vi "Playground_Variant Attributes to Cluster.vi"() -> ()   [LabVIEW 2019]
uses:
  Classes/Settings/ObjectSettings/ObjectSettings.lvclass
  subVIs/typedefs/Schedule Types/Schedule--Ramp.ctl
  <vilib>/JDP Science/JSONtext/JSONtext.lvlib
  60cf58b4-a140-46e7-9bca-05715a14d1c5.vi
  26d5b9b7-31bc-4fce-ba1d-d7f4b91fb41a.vi
  subVIs/typedefs/Schedule Types/Schedule--Constant.ctl
  6ec7998a-a771-46c5-871c-0acc70d3b499.vi
  8034bc6a-2b88-43b4-ab5e-da1cf6f0a6e7.vi
panel:
  out "<JSON> 4":string
  out "Data out":T1={"Value"=10.0}
  in  "error in (no error)":errorcluster
  in  "LUT In":variant
  out "<JSON> 2":string caption="<JSON>First JSON Value"
  out "Rest of Input String":string
  out "<JSON> 3":string caption="<JSON>"
  out "names":string[](array[string])
  out "data":string[](array[string])
  out "<JSON>":string
  out "Array":variant[](array[variant])
  out "x/y":dbl
  # "Read"
  # "JDP: 4.65363E-5"
  # "JKI: 0.0002399"
  # "Write"
  # "JDP: 3.40146E-5\nJKI: 8.64174E-5"
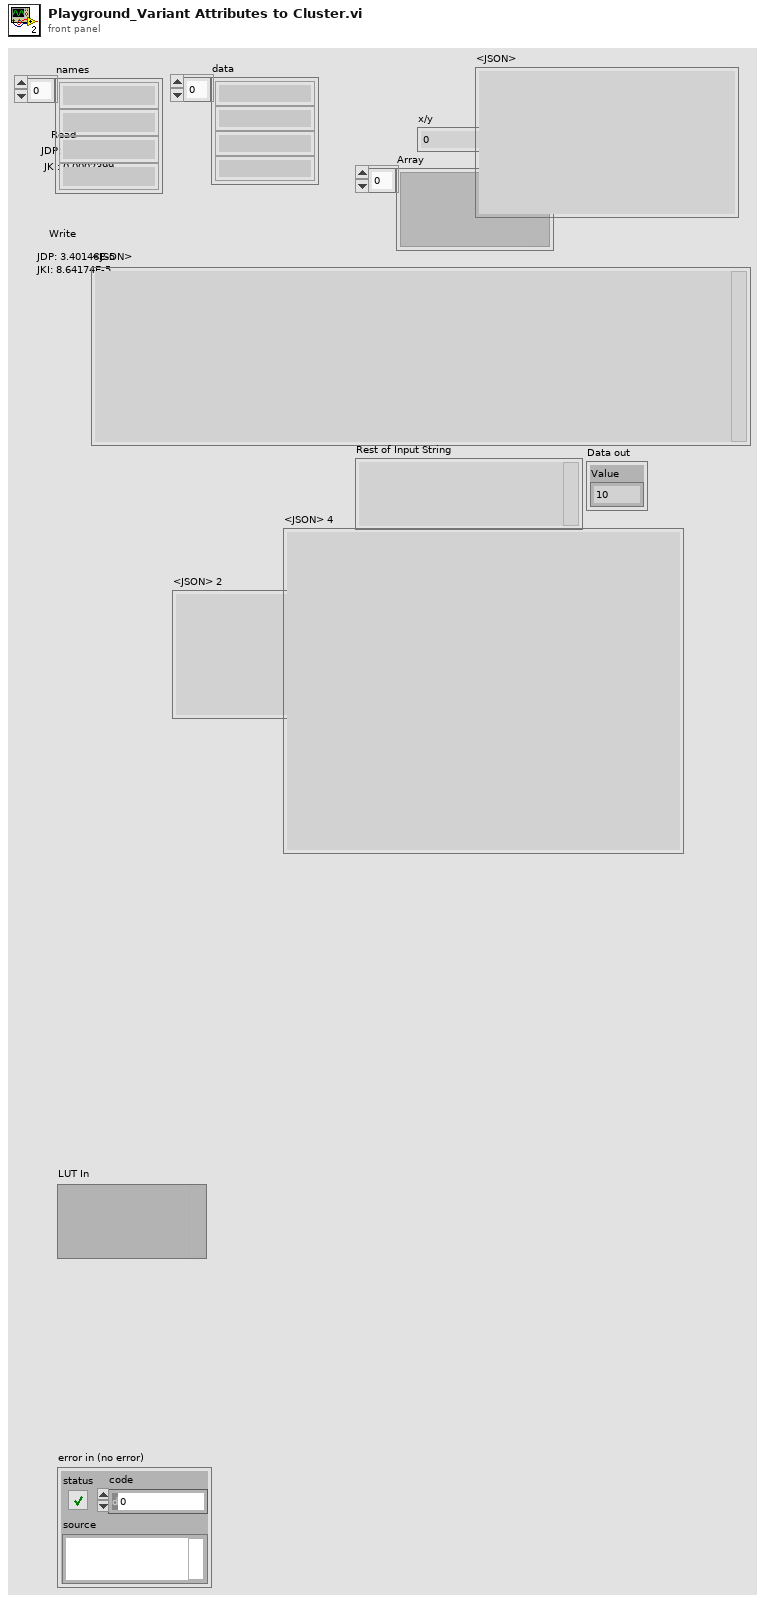
[diagram p1: front panel]
types:
  T1 = typedef "Schedule--Constant.ctl" = cluster{"Value":dbl}
  T2 = typedef "Schedule--Ramp.ctl" = cluster{"Start":dbl, "End":dbl}
  T3 = cluster{"Attribute 1":bool, "Attribute 2":string, "Attribute 3":string}
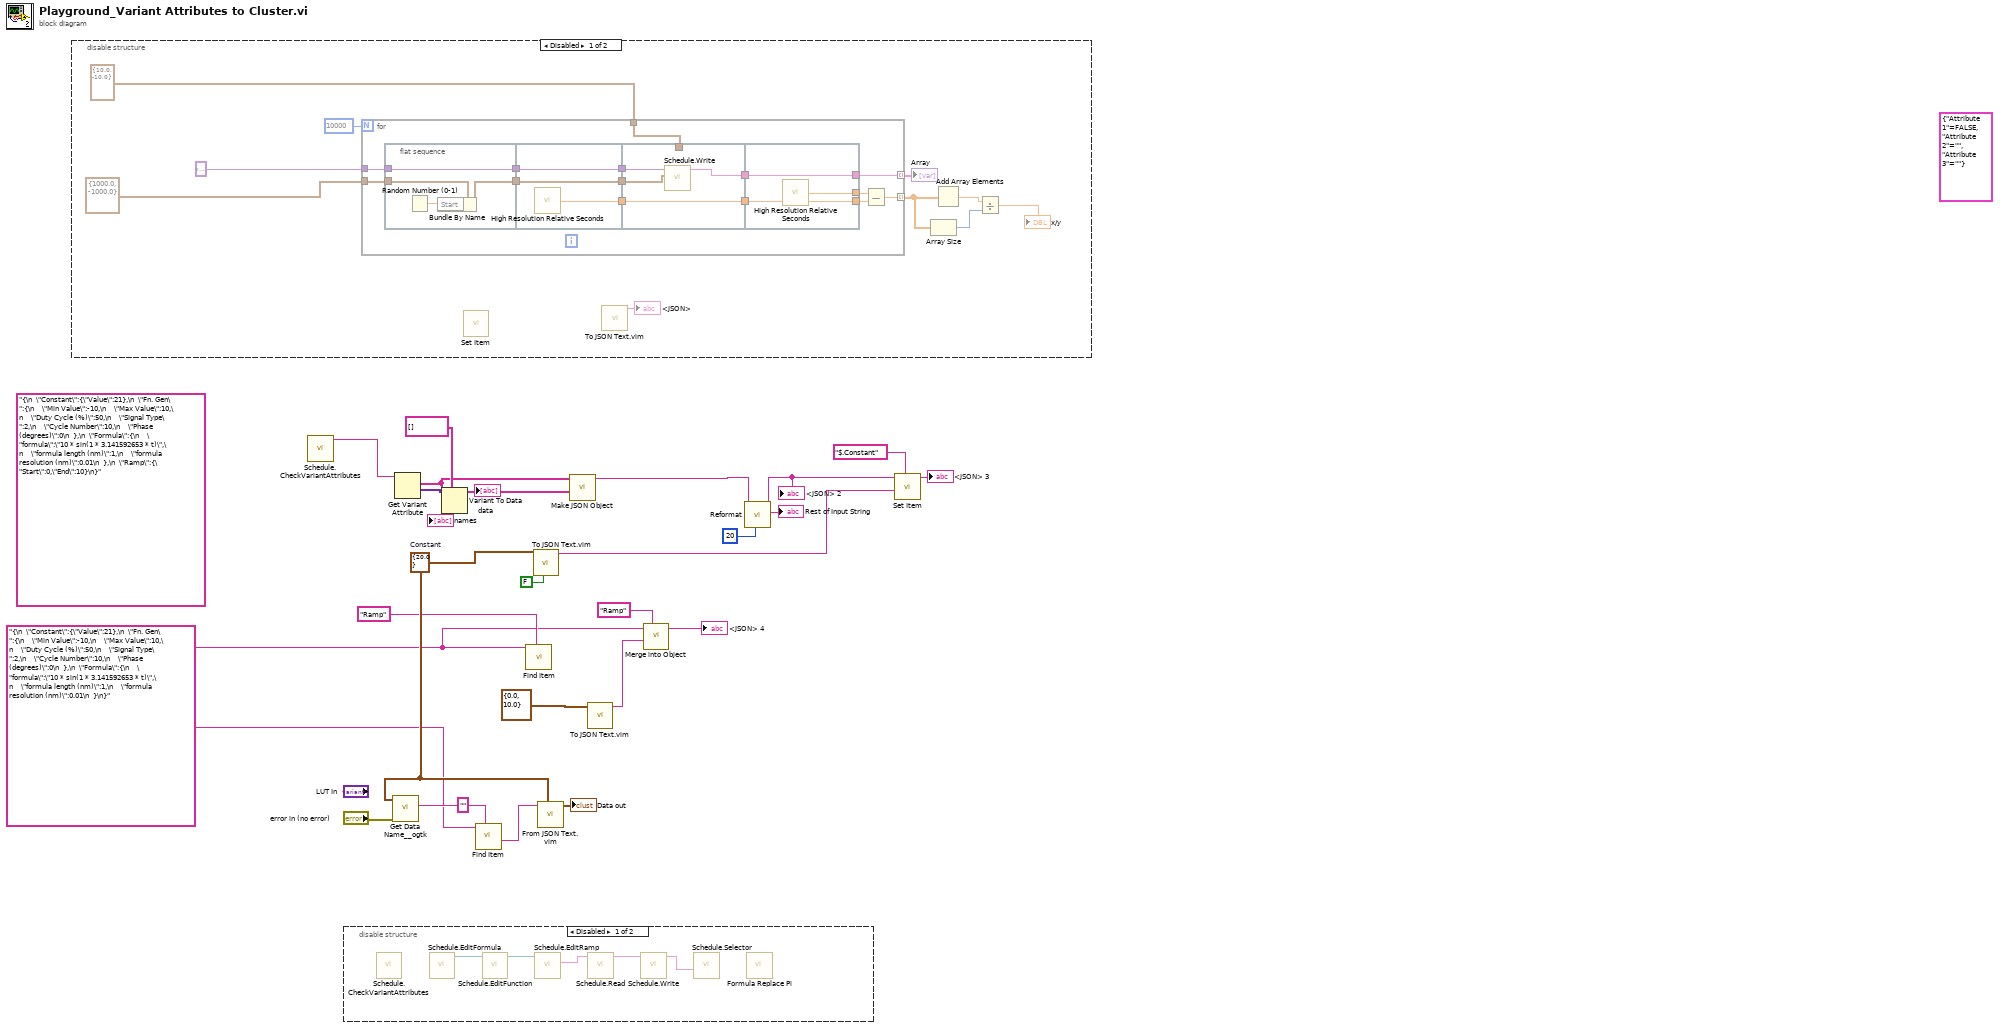
[diagram p0: block diagram]
diagram:
  (unwired) "{\n  \"Constant\":{\"Value\":21},\n  \"Fn. Gen\":{\n    \"Min Value\":-10,\n    \"Max Value\":10,\n    \"Duty Cycle (%)\":50,\n    \"Signal Type\":2,\n    \"Cycle Number\":10,\n    \"Phase (degrees)\":0\n  },\n  \"Formula\":{\n    \"formula\":\"10 * sin(1 * 3.141592653 * t)\",\n    \"formula length (nm)\":1,\n    \"formula resolution (nm)\":0.01\n  },\n  \"Ramp\":{\"Start\":0,\"End\":10}\n}" ("<JSON> 2")
  w4 = "{\n  \"Constant\":{\"Value\":21},\n  \"Fn. Gen\":{\n    \"Min Value\":-10,\n    \"Max Value\":10,\n    \"Duty Cycle (%)\":50,\n    \"Signal Type\":2,\n    \"Cycle Number\":10,\n    \"Phase (degrees)\":0\n  },\n  \"Formula\":{\n    \"formula\":\"10 * sin(1 * 3.141592653 * t)\",\n    \"formula length (nm)\":1,\n    \"formula resolution (nm)\":0.01\n  }\n}" ("<JSON> 2")
  (unwired) ""
  w10 = T1 {"Value"=20.0}  # Constant
  (unwired) T3 {"Attribute 1"=FALSE, "Attribute 2"="", "Attribute 3"=""}
  n1 = disable-structure shown="Disabled" {
    frame Disabled {
      n2 = for {
        N: 10000 -> [_]
        tunnel: T2 {"Start"=10.0, "End"=-10.0} ("Ramp") -> [w47]
        tunnel: variant ("LUT In") -> [w49]
        tunnel: [w48] -> w27 mode=indexing
        tunnel: [w40] -> w33 mode=indexing
        tunnel: T2 {"Start"=1000.0, "End"=-1000.0} ("Ramp") -> [w37]
        n3 = flat-sequence {
          tunnel: w49 -> [w53]
          tunnel: [w53] -> w39
          tunnel: [w52] -> w38
          tunnel: w37 -> [w51]
          tunnel: [w56] -> w46
          tunnel: [w55] -> w43
          tunnel: w39 -> [w56]
          tunnel: w38 -> [w54]
          tunnel: [w54] -> w36
          tunnel: w47 -> [_]
          tunnel: w46 -> [w59]
          tunnel: [w58] -> w45
          tunnel: [w60] -> w44
          tunnel: w43 -> [w60]
          tunnel: w36 -> [w57]
          tunnel: [w63] -> w48
          tunnel: w45 -> [w63]
          tunnel: [w62] -> w41
          tunnel: w44 -> [w62]
          tunnel: [w61] -> w42
          frame #0 {
            n4 = Random Number (0-1)() -> (number: 0 to 1=w50:dbl)
            n5 = Bundle By Name(cluster=w51, "Start"=w50) -> (w52:T2)
          }
          frame #1 {
            n6 = call <vilib>:"High Resolution Relative Seconds.vi"() -> ("relative seconds"=w55:dbl)
          }
          frame #2 {
            n7 = call "Schedule.Write.vi"("Data to Write"=w57, "Schedule <JSON> In"=w59) -> ("Schedule <JSON> Out"=w58:string)  [unwired: 8 in, 1 out]
          }
          frame #3 {
            n8 = call <vilib>:"High Resolution Relative Seconds.vi"() -> ("relative seconds"=w61:dbl)
          }
        }
        n9 = Subtract(x=w42, y=w41) -> (x-y=w40:dbl)
      }
      "Array" <- w27
      n10 = call <vilib>:"Set Item.vi"() -> ()  [unwired: 8 in, 3 out]
      n11 = call "To JSON Text.vim"() -> ("<JSON>"=→"<JSON>":string, "Anything"=w26:variant)  [unwired: 9 in, 1 out]
      n12 = Array Size(array=w33) -> (size(s)=w31:i32)
      n13 = Add Array Elements(numeric array=w33) -> (sum=w32:dbl)
      n14 = Divide(x=w32, y=w31) -> (x/y=→"x/y":dbl)
    }
    frame Enabled {
    }
  }
  n15 = call "Schedule.CheckVariantAttributes.vi"() -> ("Schedule <JSON> Out"=w24:string)  [unwired: 10 in, 1 out]
  n16 = disable-structure shown="Disabled" {
    frame Disabled {
      n17 = call "Schedule.CheckVariantAttributes.vi"() -> ()  [unwired: 10 in, 2 out]
      n18 = call-dynamic "Schedule.EditFormula.vi"() -> ("ObjectSettings out"=w68:refnum<class "ObjectSettings.lvclass">)  [unwired: 9 in, 2 out]
      n19 = call-dynamic "Schedule.EditFunction.vi"("ObjectSettings in"=w68) -> ("ObjectSettings out"=w67:refnum<class "ObjectSettings.lvclass">)  [unwired: 8 in, 2 out]
      n20 = call-dynamic "Schedule.EditRamp.vi"("ObjectSettings in"=w67) -> ("Settings Out"=w66:string)  [unwired: 8 in, 2 out]
      n21 = call "Schedule.Read.vi"("Schedule <JSON> In"=w66) -> ("Schedule <JSON> Out"=w65:string)  [unwired: 8 in, 2 out]
      n22 = call "Schedule.Write.vi"("Schedule <JSON> In"=w65) -> ("Schedule <JSON> Out"=w64:string)  [unwired: 9 in, 1 out]
      n23 = call-dynamic "Schedule.Selector.vi"("Settings In"=w64) -> ()  [unwired: 8 in, 3 out]
      n24 = call "Formula Replace Pi.vi"() -> ()  [unwired: 5 in, 1 out]
    }
    frame Enabled {
    }
  }
  n25 = call <userlib>:"Get Data Name__ogtk.vi"("error in (no error)"="error in (no error)", "Data"=w10) -> ("Data Name"=w9:string)  [unwired: 7 in, 2 out]
  n26 = Get Variant Attribute(Variant=w24) -> (names=w20:string[], values=w23:variant[])  [unwired: 3 in, 2 out]
  "names" <- w20
  n27 = Variant To Data(type=string[] [], Variant=w23) -> (data=w21:string[])  [unwired: 1 in, 1 out]
  "data" <- w21
  n28 = call <vilib>:"Find Item.vi"("$Path or Item Name"=w9, "JSON"=w4) -> ("<JSON>"=w8:string)  [unwired: 6 in, 3 out]
  n29 = call <vilib>:"Find Item.vi"("$Path or Item Name"="Ramp", "JSON"=w4) -> ()  [unwired: 6 in, 4 out]
  n30 = call "To JSON Text.vim"("Pretty Print?"=FALSE, "Anything"=w10) -> ("<JSON>"=w17:string)  [unwired: 8 in, 1 out]
  n31 = call "From JSON Text.vim"("Data Type and Default Value"=w10, "JSON"=w8) -> ("Data out"=→"Data out":T1)  [unwired: 8 in, 1 out]
  n32 = call <vilib>:"Make JSON Object.vi"("JSON Items"=w21, "Item Names"=w20) -> ("<JSON>"=w15:string)  [unwired: 8 in, 1 out]
  n33 = call "To JSON Text.vim"("Anything"=T2 {"Start"=0.0, "End"=10.0} ("Ramp")) -> ("<JSON>"=w3:string)  [unwired: 9 in, 1 out]
  n34 = call <vilib>:"Merge into Object.vi"("$Path or Item Name"="Ramp", "JSON Object to Merge"=w3, "JSON"=w4) -> ("<JSON>"=→"<JSON> 4":string)  [unwired: 6 in, 1 out]
  n35 = call <vilib>:"Reformat.vi"("Pretty Print Levels"=20, "JSON"=w15) -> ("Rest of Input String"=→"Rest of Input String":string, "<JSON>"=w14:string)  [unwired: 6 in, 2 out]
  "<JSON> 2" <- w14
  n36 = call <vilib>:"Set Item.vi"("$Path or Item Name"="$.Constant", "JSON to Insert"=w17, "JSON"=w14) -> ("<JSON>"=→"<JSON> 3":string)  [unwired: 5 in, 2 out]
